vi "Raw Publisher to Refnum.vi"(3 "Raw Publisher U64":u64) -> (5 "Raw Publisher Refnum":T1 {"refnum" format="%.0x"})   [LabVIEW 2021, in "Iceoryx.lvlib"]
uses:
  Iceoryx.lvlib
  Typedef/Raw Publisher Refnum.ctl
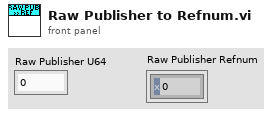
[diagram p1: front panel]
types:
  T1 = typedef "Iceoryx.lvlib/Raw Publisher Refnum.ctl" = cluster{"refnum":u64, "Raw Pub":enum8{"rawpub"}}
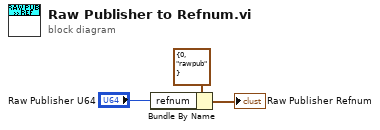
[diagram p0: block diagram]
diagram:
  n1 = Bundle By Name(cluster=T1 {"refnum"=0, "Raw Pub"=enum."rawpub"} ("Raw Publisher Refnum"), "refnum"="Raw Publisher U64") -> (→"Raw Publisher Refnum":T1)
